vi "Burst Pattern.vi"(7 "DPI Instrument Name":refnum<k15>, 8 "DUT Bring Up Pins":string[](array[string]), 9 "List-Current Measurement Pins":string[](array[string]), 10 "List-Patterns":string[](array[string]), 11 "DPE Project File Path":string) -> (0 "error out":errorcluster, 3 "Measurement Results":T1)   [LabVIEW 2025, in "Digital Pattern Sequencer.lvclass"]
uses:
  Digital Pattern Sequencer.lvclass
  Digital Pattern Sequencer.lvclass/Digital Pattern Sequencer.ctl
  <instrlib>/niDigital/niDigital.llb/niDigital Selected Function.ctl
  <instrlib>/niDCPower/nidcpower.llb/niDCPower Source Mode.ctl
  <instrlib>/niDCPower/nidcpower.llb/niDCPower Wait For Event - Event.ctl
  <instrlib>/niDCPower/nidcpower.llb/niDCPower Output Function.ctl
  Measurement Results.ctl
  <instrlib>/niDigital/niDigital.llb/niDigital Burst Pattern (Pass Fail).vi
  <instrlib>/niDCPower/nidcpower.llb/niDCPower Get Channel Name From String.vi
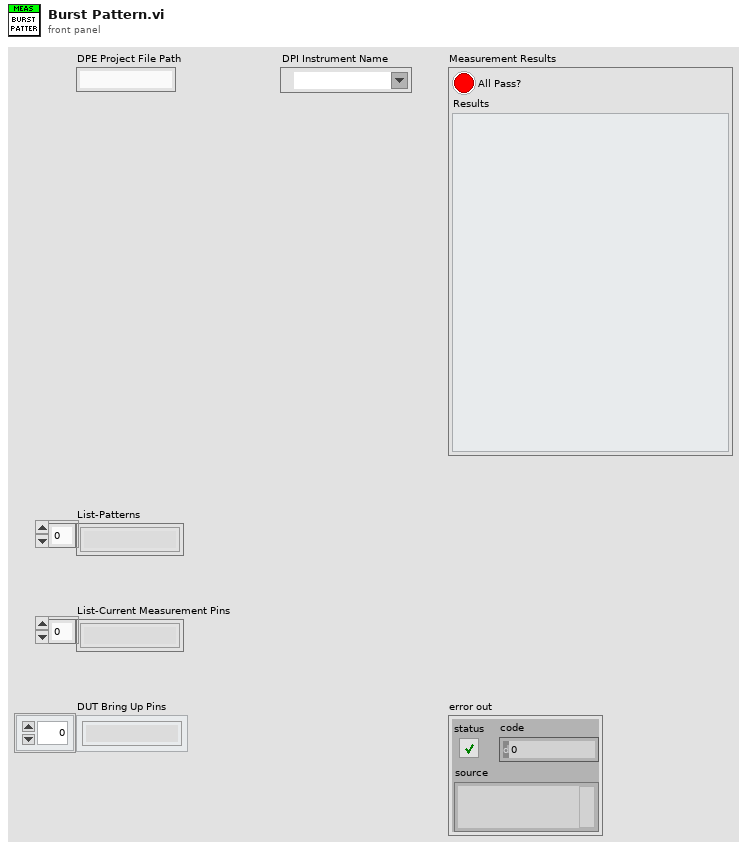
[diagram p1: front panel]
types:
  T1 = typedef "Digital Pattern Sequencer.lvclass/Measurement Results.ctl" = cluster{"All Pass?":bool, "Results":string}
  T2 = typedef "niDigital Selected Function.ctl" = i32
  T3 = typedef "niDCPower Output Function.ctl" = i32
  T4 = typedef "niDCPower Wait For Event - Event.ctl" = i32
  T5 = typedef "niDCPower Source Mode.ctl" = i32
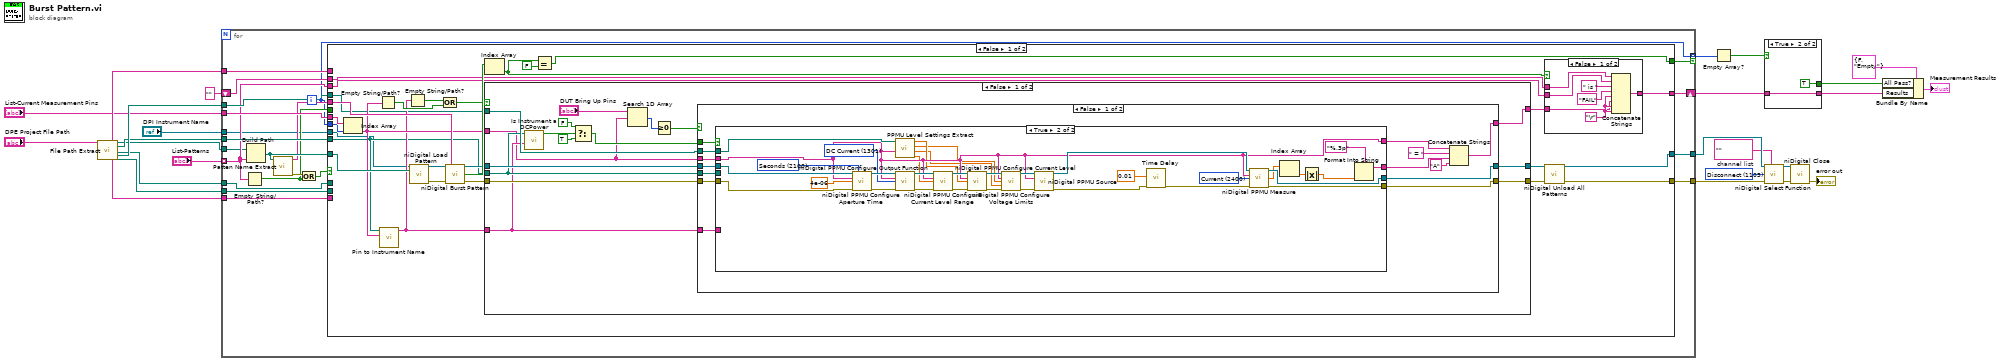
[diagram p0: block diagram]
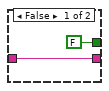
[diagram p2: hidden frame]
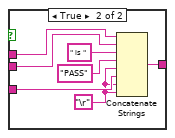
[diagram p3: hidden frame]
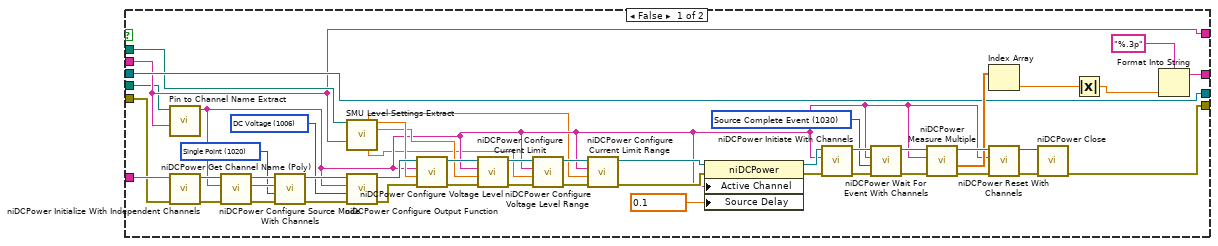
[diagram p4: hidden frame]
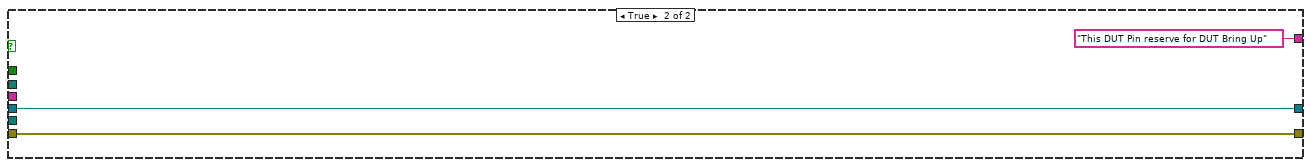
[diagram p5: hidden frame]
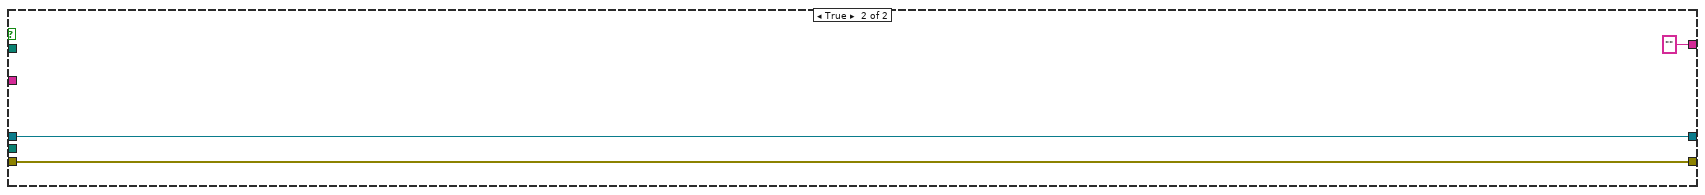
[diagram p6: hidden frame]
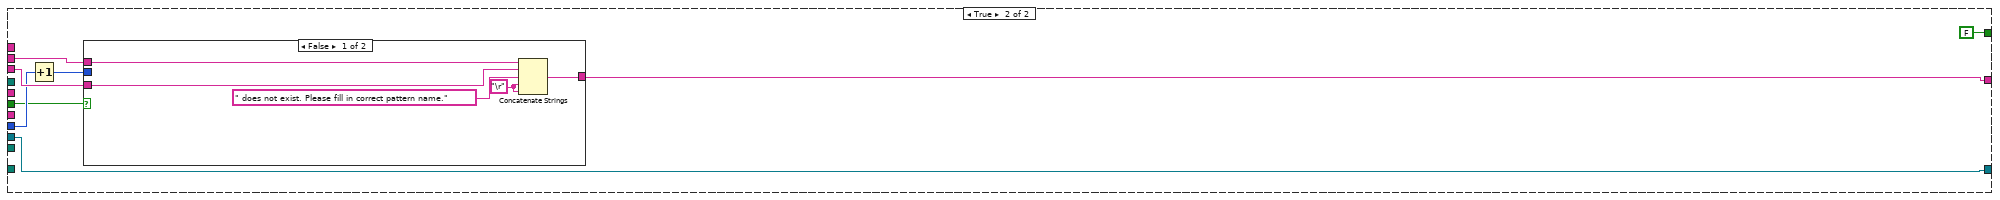
[diagram p7: hidden frame]
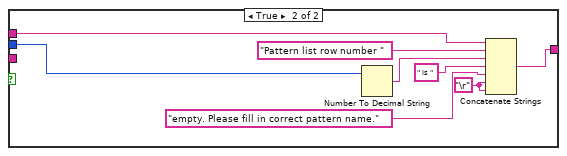
[diagram p8: hidden frame]
diagram:
  w4 = ""  # channel list
  w3 = T2 1103 items=["Digital"=1100, "PPMU"=1101, "Off"=1102, "Disconnect"=1103] ("function")
  n1 = call "File Path Extract.vi"("DPE Project File Path"="DPE Project File Path") -> ("Timing path name"=w25:string, "Level path name"=w26:string, "DPE Project Path"=w20:path, ".pinmap file path"=w21:path, ".digitiming file path"=w22:path, ".digilevels file path"=w23:path, ".spec file path"=w24:path)  [unwired: 10 in, 2 out]
  n2 = for {
    tunnel: w25 -> [w47]
    tunnel: w26 -> [w46]
    tunnel: w21 -> [w42]
    tunnel: w24 -> [w45]
    tunnel: w23 -> [w44]
    tunnel: w22 -> [w43]
    tunnel: "List-Patterns" -> [w39] mode=indexing
    tunnel: w20 -> [w38]
    tunnel: "List-Current Measurement Pins" -> [w41]
    shift-right: [w32] -> w16
    shift-left: "" -> [w40]
    tunnel: [w31] -> w17 mode=indexing if=w30
    tunnel: "DPI Instrument Name" -> [w29]
    tunnel: [w28] -> w5
    tunnel: [w27] -> w2
    i -> [w31]
    n3 = Empty String/Path?(string/path=w39) -> (empty?=w33:bool)
    n4 = Build Path(base path=w38, name or relative path=w39) -> (appended path=w36:path)
    n5 = call "Patten Name Extract.vi"("Digipat source file"=w36) -> ("error out"=w34:errorcluster, "pattern name"=w35:string)  [unwired: 9 in]
    n6 = Or(x=w34, y=w33) -> (x .or. y?=w37:bool)
    n7 = case shown="False" w37 {
      tunnel: w47 -> [_ _]
      tunnel: w46 -> [_ _]
      tunnel: w45 -> [_ _]
      tunnel: w44 -> [w56 _]
      tunnel: w43 -> [_ _]
      tunnel: w42 -> [w57 _]
      tunnel: w41 -> [w70 _]
      tunnel: w31 -> [w66 w213]
      tunnel: w39 -> [w69 w214]
      tunnel: [w68 w210] -> w32
      tunnel: w40 -> [w67 w209]
      tunnel: w36 -> [w61 _]
      tunnel: w35 -> [w60 _]
      tunnel: w33 -> [_ w211]
      tunnel: [w53 FALSE] -> w30
      tunnel: w29 -> [w52 w207]
      tunnel: [w50 w207] -> w28
      tunnel: [w48 _] -> w27
      frame False {
        n8 = Index Array(array=w70, index=w66) -> (element=w59:string)
        n9 = Empty String/Path?(string/path=w59) -> (empty?=w62:bool)
        n10 = call "Pin to Instrument Name.vi"(".pinmap File Path"=w57, "Pin Name"=w59) -> ("Instrument Name"=w58:string)  [unwired: 8 in]
        n11 = Empty String/Path?(string/path=w58) -> (empty?=w64:bool)
        n12 = call <instrlib>:"niDigital Load Pattern.vi"("instrument handle"=w52, "pattern file"=w61) -> ("instrument handle out"=w75:refnum<k15>, "error out"=w74:errorcluster)  [unwired: 12 in]
        n13 = Or(x=w64, y=w62) -> (x .or. y?=w63:bool)
        n14 = call-poly <instrlib>:"niDigital Burst Pattern.vi"("instrument handle"=w75, "start label"=w60, "error in"=w74) -> ("instrument handle out"=w72:refnum<k15>, "pass"=w73:bool[], "error out"=w71:errorcluster)  [unwired: 10 in]
        n15 = Index Array(array=w73) -> (element=w55:bool)  [unwired: 1 in]
        n16 = case shown="False" w63 {
          tunnel: w72 -> [w105 w205]
          tunnel: w71 -> [w104 w206]
          tunnel: [w103 w205] -> w51
          tunnel: [w102 w206] -> w49
          tunnel: [w101 ""] -> w65
          tunnel: w59 -> [w92 _]
          tunnel: w58 -> [w94 _]
          tunnel: w57 -> [w99 _]
          tunnel: w56 -> [w100 _]
          frame False {
            n17 = call "Is Instrument a DCPower.vi"("Instrument Name"=w94, ".pinmap File Path"=w99) -> ("DCPower?"=w97:bool)  [unwired: 9 in]
            n18 = Select(t=FALSE, s=w97, f=TRUE) -> (s? t:f=w98:bool)
            n19 = Search 1D Array(1D array="DUT Bring Up Pins", element=w92) -> (index of element=w90:i32)  [unwired: 1 in]
            n20 = Greater Or Equal To 0?(x=w90) -> (x >= 0?=w91:bool)
            n21 = case shown="False" w91 {
              tunnel: w105 -> [w119 w203]
              tunnel: w104 -> [w118 w202]
              tunnel: [w117 w203] -> w103
              tunnel: [w116 w202] -> w102
              tunnel: w92 -> [w115 _]
              tunnel: [w112 "This DUT Pin reserve for DUT Bring Up"] -> w101
              tunnel: w100 -> [w109 _]
              tunnel: w99 -> [w108 _]
              tunnel: w98 -> [w107 _]
              tunnel: w94 -> [w106 _]
              frame False {
                n22 = case shown="True" w107 {
                  tunnel: w119 -> [w133 w186]
                  tunnel: w118 -> [w122 w185]
                  tunnel: [w133 w184] -> w117
                  tunnel: [w132 w183] -> w116
                  tunnel: w115 -> [w125 w172]
                  tunnel: w106 -> [w135 _]
                  tunnel: [w134 w181] -> w113
                  tunnel: [w125 w172] -> w111
                  tunnel: w109 -> [w128 w173]
                  tunnel: w108 -> [w124 _]
                  frame False {
                    w136 = T3 1006 items=["DC Voltage"=1006, "DC Current"=1007, "Pulse Voltage"=1049, "Pulse Current"=1050] ("output function")
                    w139 = T4 1030 items=["Source Complete Event"=1030, "Measure Complete Event"=1031, "Sequence Iteration Complete Event"=1032, "Sequence Engine Done Event"=1033] ("event")
                    w138 = T5 1020 items=["Single Point"=1020, "Sequence"=1021] ("source mode")
                    n23 = call "Pin to Channel Name Extract.vi"(".pinmap File Path"=w124, "Pin Name"=w125) -> ("Channel"=w123:string)  [unwired: 8 in]
                    n24 = call <instrlib>:"niDCPower Initialize With Independent Channels.vi"("error in (no error)"=w122, "resource name"=w135) -> ("error out"=w163:errorcluster, "instrument handle out"=w144:refnum<k15>)  [unwired: 8 in]
                    n25 = call-poly <instrlib>:"niDCPower Get Channel Name (Poly).vi"("error in (no error)"=w163, "index"=w123, "instrument handle"=w144) -> ("error out"=w164:errorcluster, "name"=w165:string, "instrument handle out"=w162:refnum<k15>)  [unwired: 6 in]
                    n26 = call <instrlib>:"niDCPower Configure Source Mode With Channels.vi"("error in (no error)"=w164, "source mode"=w138, "channel name"=w165, "instrument handle"=w162) -> ("error out"=w145:errorcluster, "instrument handle out"=w146:refnum<k15>)  [unwired: 6 in]
                    n27 = call "SMU Level Settings Extract.vi"(".digilevel File Path"=w128, "Pin Name"=w125) -> ("IRange"=w120:dbl, "Vf"=w127:dbl, "Ic"=w126:dbl, "VRange"=w121:dbl)  [unwired: 7 in, 3 out]
                    n28 = call <instrlib>:"niDCPower Configure Output Function.vi"("error in (no error)"=w145, "output function"=w136, "channel name"=w123, "instrument handle"=w146) -> ("error out"=w161:errorcluster, "instrument handle out"=w160:refnum<k15>)  [unwired: 6 out]
                    n29 = call <instrlib>:"niDCPower Configure Voltage Level.vi"("error in (no error)"=w161, "voltage level"=w127, "channel name"=w123, "instrument handle"=w160) -> ("error out"=w141:errorcluster, "instrument handle out"=w140:refnum<k15>)  [unwired: 6 out]
                    n30 = call <instrlib>:"niDCPower Configure Current Limit.vi"("error in (no error)"=w141, "current limit"=w126, "channel name"=w123, "instrument handle"=w140) -> ("error out"=w147:errorcluster, "instrument handle out"=w148:refnum<k15>)  [unwired: 1 in, 5 out]
                    n31 = call <instrlib>:"niDCPower Configure Voltage Level Range.vi"("error in (no error)"=w147, "voltage level range"=w121, "channel name"=w123, "instrument handle"=w148) -> ("error out"=w149:errorcluster, "instrument handle out"=w150:refnum<k15>)  [unwired: 6 out]
                    n32 = call <instrlib>:"niDCPower Configure Current Limit Range.vi"("error in (no error)"=w149, "current limit range"=w120, "channel name"=w123, "instrument handle"=w150) -> ("error out"=w155:errorcluster, "instrument handle out"=w152:refnum<k15>)  [unwired: 6 out]
                    n33 = property class="niDCPower"(reference=w152, error in=w155, "Active Channel"=w123, "Source Delay"=0.1 ("Source Delay (Sec)")) -> (reference out=w153:refnum<k15>, error out=w154:errorcluster)
                    n34 = call <instrlib>:"niDCPower Initiate With Channels.vi"("error in (no error)"=w154, "channel name"=w123, "instrument handle"=w153) -> ("error out"=w158:errorcluster, "instrument handle out"=w156:refnum<k15>)  [unwired: 7 in]
                    n35 = call <instrlib>:"niDCPower Wait For Event With Channels.vi"("error in (no error)"=w158, "event"=w139, "channel name"=w123, "instrument handle"=w156) -> ("error out"=w159:errorcluster, "instrument handle out"=w157:refnum<k15>)  [unwired: 6 in]
                    n36 = call <instrlib>:"niDCPower Measure Multiple.vi"("error in (no error)"=w159, "channel name"=w123, "instrument handle"=w157) -> ("error out"=w167:errorcluster, "current measurements"=w151:dbl[], "instrument handle out"=w166:refnum<k15>)  [unwired: 6 out]
                    n37 = Index Array(array=w151) -> (element=w130:dbl)  [unwired: 1 in]
                    n38 = call <instrlib>:"niDCPower Reset With Channels.vi"("error in (no error)"=w167, "channel name"=w123, "instrument handle"=w166) -> ("error out"=w143:errorcluster, "instrument handle out"=w142:refnum<k15>)  [unwired: 7 in]
                    n39 = call <instrlib>:"niDCPower Close.vi"("error in (no error)"=w143, "instrument handle"=w142) -> ("error out"=w132:errorcluster)  [unwired: 9 out]
                    n40 = Absolute Value(x=w130) -> (abs(x)=w129:dbl)
                    n41 = Format Into String(format string="%.3p", w129) -> (resulting string=w134:string)  [unwired: 2 in, 1 out]
                  }
                  frame True {
                    w198 = u16 2400 items=["Voltage"=2401, "Current"=2400] ("measurement type")
                    w199 = u16 2100 items=["Seconds"=2100] ("aperture time units")
                    w190 = u16 1301 items=["DC Voltage"=1300, "DC Current"=1301] ("output function")
                    n42 = call <instrlib>:"niDigital PPMU Configure Aperture Time.vi"("instrument handle"=w186, "aperture time units"=w199, "channel list"=w172, "aperture time"=4e-06, "error in"=w185) -> ("instrument handle out"=w197:refnum<k15>, "error out"=w196:errorcluster)  [unwired: 9 in]
                    n43 = call "PPMU Level Settings Extract.vi"("Pin Name"=w172, ".digilevel File Path"=w173) -> ("IRange"=w171:dbl, "Vcl"=w168:dbl, "Vch"=w169:dbl, "If"=w170:dbl)  [unwired: 5 in, 1 out]
                    n44 = call <instrlib>:"niDigital PPMU Configure Output Function.vi"("instrument handle"=w197, "channel list"=w172, "output function"=w190, "error in"=w196) -> ("instrument handle out"=w192:refnum<k15>, "error out"=w189:errorcluster)  [unwired: 10 in]
                    n45 = call <instrlib>:"niDigital PPMU Configure Current Level Range.vi"("instrument handle"=w192, "channel list"=w172, "current level range (A)"=w171, "error in"=w189) -> ("instrument handle out"=w191:refnum<k15>, "error out"=w188:errorcluster)  [unwired: 10 in]
                    n46 = call <instrlib>:"niDigital PPMU Configure Current Level.vi"("instrument handle"=w191, "channel list"=w172, "current level (A)"=w170, "error in"=w188) -> ("instrument handle out"=w179:refnum<k15>, "error out"=w177:errorcluster)  [unwired: 10 in]
                    n47 = call <instrlib>:"niDigital PPMU Configure Voltage Limits.vi"("instrument handle"=w179, "channel list"=w172, "voltage limit high (V)"=w169, "voltage limit low (V)"=w168, "error in"=w177) -> ("instrument handle out"=w178:refnum<k15>, "error out"=w176:errorcluster)  [unwired: 9 in]
                    n48 = call <instrlib>:"niDigital PPMU Source.vi"("instrument handle"=w178, "channel list"=w172, "error in"=w176) -> ("instrument handle out"=w200:refnum<k15>, "error out"=w187:errorcluster)  [unwired: 11 in]
                    n49 = call "Time Delay"("error in (no error)"=w187, "Delay Time (s)"=0.01 ("settling time (s)")) -> ("error out"=w193:errorcluster)  [unwired: 9 in]
                    n50 = call <instrlib>:"niDigital PPMU Measure.vi"("instrument handle"=w200, "channel list"=w172, "measurement type"=w198, "error in"=w193) -> ("instrument handle out"=w184:refnum<k15>, "measurements"=w182:dbl[], "error out"=w183:errorcluster)  [unwired: 9 in]
                    n51 = Index Array(array=w182) -> (element=w175:dbl)  [unwired: 1 in]
                    n52 = Absolute Value(x=w175) -> (abs(x)=w174:dbl)
                    n53 = Format Into String(format string="%.3p", w174) -> (resulting string=w181:string)  [unwired: 2 in, 1 out]
                  }
                }
                n54 = Concatenate Strings(w111, " = " ("string"), w113, "A" ("string")) -> (w112:string)
              }
              frame True {
              }
            }
          }
          frame True {
          }
        }
        n55 = Equal?(x=w55, y=FALSE) -> (x = y?=w53:bool)
        n56 = case shown="False" w55 {
          tunnel: w69 -> [w78 w89]
          tunnel: [w76 w87] -> w68
          tunnel: w67 -> [w79 w86]
          tunnel: w65 -> [w77 w85]
          frame False {
            w81 = "\r"
            n57 = Concatenate Strings(w79, w78, " is " ("string"), "FAIL", w81, w77, w81, w81) -> (w76:string)
          }
          frame True {
            w84 = "\r"
            n58 = Concatenate Strings(w86, w89, " is " ("string"), "PASS", w84, w85, w84, w84) -> (w87:string)
          }
        }
        n59 = call <instrlib>:"niDigital Unload All Patterns.vi"("instrument handle"=w51, "error in"=w49) -> ("instrument handle out"=w50:refnum<k15>, "error out"=w48:errorcluster)  [unwired: 12 in]
      }
      frame True {
        n60 = Increment(x=w213) -> (x+1=w212:i32)
        n61 = case shown="False" w211 {
          tunnel: w214 -> [w219 _]
          tunnel: w212 -> [_ w225]
          tunnel: [w216 w221] -> w210
          tunnel: w209 -> [w215 w220]
          frame False {
            w217 = "\r"
            n62 = Concatenate Strings(w215, w219, " does not exist. Please fill in correct pattern name." ("string"), w217, w217) -> (w216:string)
          }
          frame True {
            w222 = "\r"
            n63 = Number To Decimal String(number=w225) -> (decimal integer string=w224:string)  [unwired: 1 in]
            n64 = Concatenate Strings(w220, "Pattern list row number " ("string"), w224, " is " ("string"), "empty. Please fill in correct pattern name." ("string"), w222, w222) -> (w221:string)
          }
        }
      }
    }
  }
  n65 = Empty Array?(array=w17) -> (empty?=w18:bool)
  n66 = case shown="True" w18 {
    tunnel: [FALSE TRUE] -> w13
    tunnel: w16 -> [w228 w230]
    tunnel: [w228 w230] -> w12
    frame False {
    }
    frame True {
    }
  }
  n67 = call <instrlib>:"niDigital Select Function.vi"("instrument handle"=w5, "channel list"=w4, "function"=w3, "error in"=w2) -> ("instrument handle out"=w6:refnum<k15>, "error out"=w7:errorcluster)  [unwired: 10 in]
  n68 = call <instrlib>:"niDigital Close.vi"("instrument handle"=w6, "error in"=w7) -> ("error out"=→"error out":errorcluster)  [unwired: 13 in]
  n69 = Bundle By Name(cluster=T1 {"All Pass?"=FALSE, "Results"="Empty"} ("Measurement Results"), "All Pass?"=w13, "Results"=w12) -> (→"Measurement Results":T1)
